vi "ReversedEngineering GetDepNodeIndex.vi"(1 "classInfo":T1, 2 "classInfoArray":T1[](array[typedef]), 3 "AllNodes":refnum<class "AbstractNode.lvclass">[](array[class]), 5 "error in (no error)":errorcluster) -> (11 "depNodes":i32[](array[numeric]), 13 "noOfAgg":i32[](array[numeric]), 14 "InterfaceNodes":i32[](array[numeric]), 15 "inheritanceNode":i32, 16 "compAggNodes":i32[](array[numeric]), 17 "noOfCompAgg":i32[](array[numeric]), 18 "aggNodes":i32[](array[numeric]), 19 "error out":errorcluster)   [LabVIEW 2020]
uses:
  <resource>/Framework/Providers/Open_GDS/UML/ReversedEngineering/ReversedEngineering ClassInfoType.ctl
  <resource>/Framework/Providers/Open_GDS/ClassProviders/Common/CommonVIs/CommonVIs_VisibilityType.ctl
  <resource>/Framework/Providers/Open_GDS/ClassProviders/Common/CommonVIs/CommonVIs_AttributeInfoType.ctl
  <resource>/Framework/Providers/Open_GDS/ClassProviders/Common/CommonVIs/CommonVIs_AttributeDataType.ctl
  <resource>/Framework/Providers/Open_GDS/UML/ReversedEngineering/ReversedEngineering_ClassDependencyDetailsType.ctl
  <resource>/Framework/Providers/Open_GDS/ClassProviders/Common/ScriptingFunctions/SubVIs/Scripting_ViDependencyType.ctl
  <resource>/Framework/Providers/Open_GDS/UML/AbstractNode_class/AbstractNode.lvclass
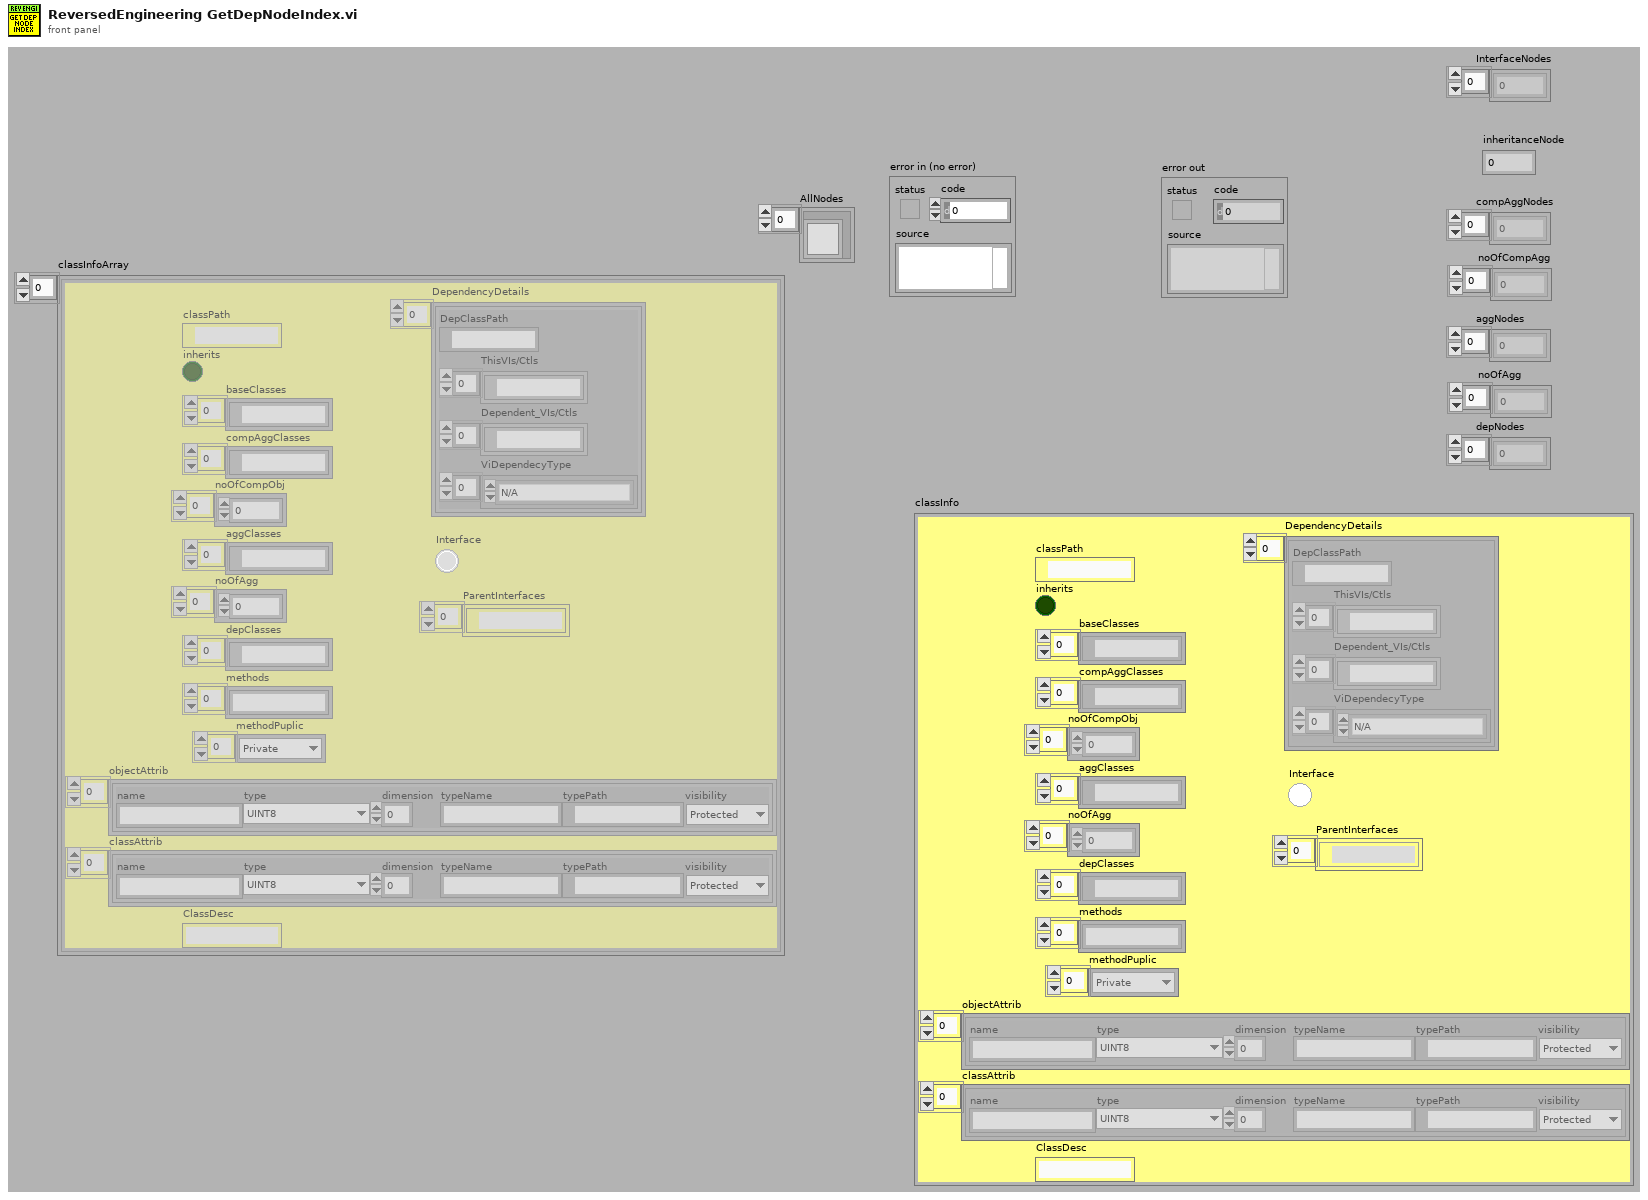
[diagram p1: front panel]
types:
  T1 = typedef "ReversedEngineering ClassInfoType.ctl" = cluster{"classPath":path, "inherits":bool, "baseClasses":path[], "compAggClasses":path[], "noOfCompObj":i32[], "aggClasses":path[], "noOfAgg":i32[], "depClasses":path[], "methods":string[], "methodPuplic":T2[], "objectAttrib":T3[], "classAttrib":T3[], "ClassDesc":string, "DependencyDetails":T5[], "Interface":bool, "ParentInterfaces":path[]}
  T2 = typedef "CommonVIs_VisibilityType.ctl" = enum16{"Public", "Private", "Protected"}
  T3 = typedef "CommonVIs_AttributeInfoType.ctl" = cluster{"name":string, "type":T4, "dimension":i32, "typeName":string, "typePath":path, "visibility":T2}
  T4 = typedef "CommonVIs_AttributeDataType.ctl" = enum16{"UINT8", "INT8", "UINT16", "INT16", "UINT32", "INT32", "UINT64", "INT64", "SGL", "DBL", "EXT", "CSG", "CDB", "CXT", "TimeStamp", "STRING", "PATH", "BOOL", "ENUM", "RefNum", "VIRefNum", "LabVIEW Class", "Cluster", "Variant", "TypeDef", "Waveform", "LabVIEW Object", "Other", "void", "Set", "Map"}
  T5 = typedef "ReversedEngineering_ClassDependencyDetailsType.ctl" = cluster{"DepClassPath":path, "ThisVIs/Ctls":path[], "Dependent_VIs/Ctls":path[], "ViDependecyType":T6[]}
  T6 = typedef "Scripting_ViDependencyType.ctl" = enum16{"N/A", "Launches"}
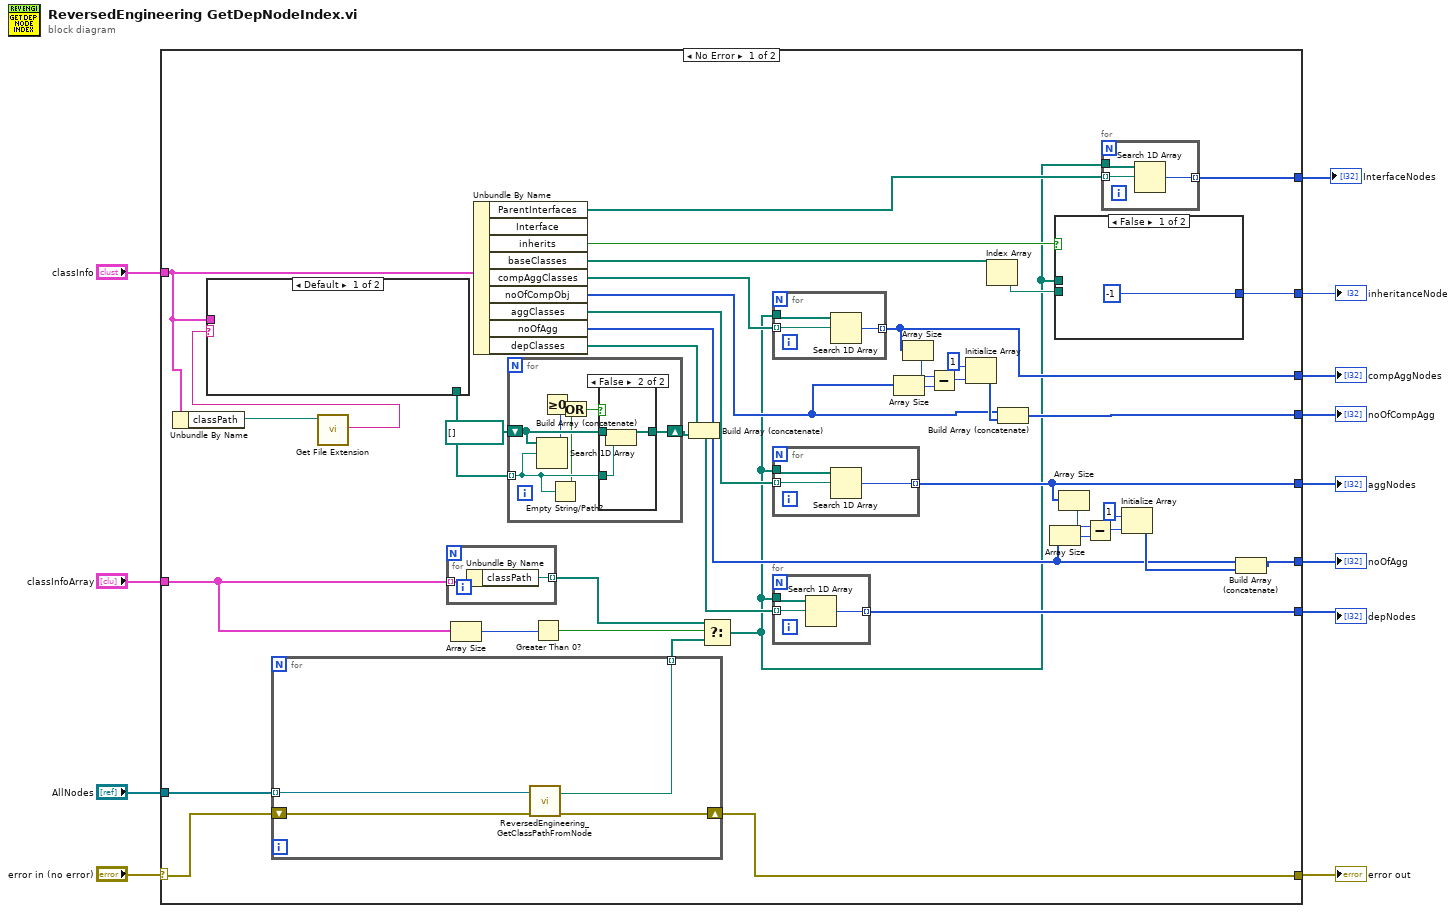
[diagram p0: block diagram]
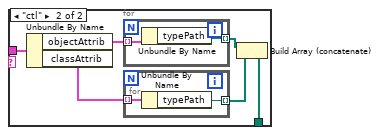
[diagram p2: hidden frame]
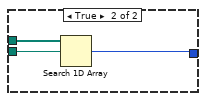
[diagram p4: hidden frame]
diagram:
  n1 = case shown="No Error" "error in (no error)" {
    selector: "error in (no error)" -> [w43 w98]
    tunnel: [w42 w98] -> w12
    tunnel: "classInfo" -> [w35 _]
    tunnel: "classInfoArray" -> [w48 _]
    tunnel: [w53 _] -> w8
    tunnel: [w32 _] -> w7
    tunnel: [w28 _] -> w6
    tunnel: [w19 _] -> w5
    tunnel: [w18 _] -> w4
    tunnel: [w49 _] -> w3
    tunnel: "AllNodes" -> [w44 _]
    tunnel: [w13 _] -> w1
    frame No Error {
      n2 = Unbundle By Name(w35) -> ("classPath"=w34:path)
      n3 = for {
        tunnel: w44 -> [w82] mode=indexing
        shift-right: [w80] -> w42
        shift-left: w43 -> [w81]
        tunnel: [w79] -> w41 mode=indexing
        n4 = call <resource>:"ReversedEngineering_GetClassPathFromNode.vi"("reference"=w82, "error IO"=w81) -> ("Path"=w79:path, "error out"=w80:errorcluster)  [unwired: 2 in, 14 out]
      }
      n5 = call <vilib>:"Get File Extension.vi"("file"=w34) -> ("lowercase file extension"=w33:string)  [unwired: 1 in, 9 out]
      n6 = case shown="Default" w33 {
        tunnel: [_ w59] -> w40
        tunnel: w35 -> [_ w58]
        frame Default {
        }
        frame "ctl" {
          n7 = Unbundle By Name(w58) -> ("objectAttrib"=w63:T3[], "classAttrib"=w62:T3[])
          n8 = for {
            tunnel: w63 -> [w67] mode=indexing
            tunnel: [w66] -> w61 mode=indexing
            n9 = Unbundle By Name(w67) -> ("typePath"=w66:path)
          }
          n10 = for {
            tunnel: w62 -> [w65] mode=indexing
            tunnel: [w64] -> w60 mode=indexing
            n11 = Unbundle By Name(w65) -> ("typePath"=w64:path)
          }
          n12 = Build Array (concatenate)(w61, w60) -> (w59:path[])
        }
      }
      n13 = for {
        tunnel: w48 -> [w97] mode=indexing
        tunnel: [w96] -> w45 mode=indexing
        n14 = Unbundle By Name(w97) -> ("classPath"=w96:path)
      }
      n15 = Array Size(array=w48) -> (size(s)=w47:i32)
      n16 = Unbundle By Name(w35) -> ("ParentInterfaces"=w15:path[], "inherits"=w54:bool, "baseClasses"=w16:path[], "compAggClasses"=w51:path[], "noOfCompObj"=w25:i32[], "aggClasses"=w50:path[], "noOfAgg"=w17:i32[], "depClasses"=w38:path[])  [unwired: 1 out]
      n17 = for {
        tunnel: w40 -> [w71] mode=indexing
        shift-right: [w74] -> w37
        shift-left: path[] [] -> [w73]
        n18 = Search 1D Array(1D array=w73, element=w71) -> (index of element=w72:i32)  [unwired: 1 out]
        n19 = Greater Or Equal To 0?(x=w72) -> (x >= 0?=w70:bool)
        n20 = Empty String/Path?(string/path=w71) -> (empty?=w69:bool)
        n21 = Or(x=w70, y=w69) -> (x .or. y?=w68:bool)
        n22 = case shown="False" w68 {
          tunnel: w71 -> [_ w78]
          tunnel: [w75 w76] -> w74
          tunnel: w73 -> [w75 w77]
          frame True {
          }
          frame False {
            n23 = Build Array (concatenate)(w77, w78) -> (w76:path[])
          }
        }
      }
      n24 = Greater Than 0?(x=w47) -> (x > 0?=w46:bool)
      n25 = Build Array (concatenate)(w38, w37) -> (w36:path[])
      n26 = Select(t=w45, s=w46, f=w41) -> (s? t:f=w14:path[])
      n27 = for {
        tunnel: w51 -> [w90] mode=indexing
        tunnel: w14 -> [w91]
        tunnel: [w89] -> w32 mode=indexing
        n28 = Search 1D Array(1D array=w91, element=w90) -> (index of element=w89:i32)  [unwired: 1 out]
      }
      n29 = for {
        tunnel: w50 -> [w87] mode=indexing
        tunnel: w14 -> [w88]
        tunnel: [w86] -> w19 mode=indexing
        n30 = Search 1D Array(1D array=w88, element=w87) -> (index of element=w86:i32)  [unwired: 1 out]
      }
      n31 = for {
        tunnel: w36 -> [w84] mode=indexing
        tunnel: w14 -> [w85]
        tunnel: [w83] -> w49 mode=indexing
        n32 = Search 1D Array(1D array=w85, element=w84) -> (index of element=w83:i32)  [unwired: 1 out]
      }
      n33 = Array Size(array=w25) -> (size(s)=w30:i32)
      n34 = Array Size(array=w32) -> (size(s)=w31:i32)
      n35 = Subtract(x=w31, y=w30) -> (x-y=w29:i32)
      n36 = Initialize Array(1 ("Numeric"), w29) -> (w27:i32[])
      n37 = Index Array(array=w16) -> (element=w52:path)  [unwired: 1 in]
      n38 = Build Array (concatenate)(w25, w27) -> (w28:i32[])
      n39 = Array Size(array=w17) -> (size(s)=w21:i32)
      n40 = case shown="False" w54 {
        tunnel: [-1 ("inheritanceNode") w93] -> w53
        tunnel: w14 -> [_ w95]
        tunnel: w52 -> [_ w94]
        frame False {
        }
        frame True {
          n41 = Search 1D Array(1D array=w95, element=w94) -> (index of element=w93:i32)  [unwired: 1 out]
        }
      }
      n42 = Array Size(array=w19) -> (size(s)=w20:i32)
      n43 = Subtract(x=w20, y=w21) -> (x-y=w22:i32)
      n44 = for {
        tunnel: w15 -> [w56] mode=indexing
        tunnel: w14 -> [w57]
        tunnel: [w55] -> w13 mode=indexing
        n45 = Search 1D Array(1D array=w57, element=w56) -> (index of element=w55:i32)  [unwired: 1 out]
      }
      n46 = Initialize Array(1 ("Numeric"), w22) -> (w23:i32[])
      n47 = Build Array (concatenate)(w17, w23) -> (w18:i32[])
    }
    frame Error {
    }
  }
  "error out" <- w12
  "compAggNodes" <- w7
  "inheritanceNode" <- w8
  "noOfCompAgg" <- w6
  "noOfAgg" <- w4
  "aggNodes" <- w5
  "depNodes" <- w3
  "InterfaceNodes" <- w1
